vi "getSerializedData.vi"(0 "reference in":refnum<class "DQMHModuleNode.lvclass">, 5 "error in (no error)":errorcluster) -> (14 "reference out":refnum<class "DQMHModuleNode.lvclass">, 15 "parent":refnum<class "AbstractNode.lvclass">, 16 "children":refnum<class "AbstractNode.lvclass">[](array[class]), 17 "xmlOut":string, 19 "error out":errorcluster)   [LabVIEW 2020, in "DQMHModuleNode.lvclass"]
doc: "Gets data to store"
uses:
  <resource>/Framework/Providers/Open_GDS/UML/DQMHModuleNode_class/DQMHModuleNode.lvclass
  C:/Program Files (x86)/National Instruments/LabVIEW 2020/resource/Framework/Providers/Open_GDS/UML/AbstractNode_class/AbstractNode.lvclass
  C:/Program Files (x86)/National Instruments/LabVIEW 2020/resource/Framework/Providers/Open_GDS/UML/RectangularNode_class/RectangularNode.lvclass
  <resource>/Framework/Providers/Open_GDS/UML/AbstractNode_class/AbstractNode.lvclass
  <resource>/Framework/Providers/Open_GDS/UML/MultiLineString_class/MultiLineString.lvclass
  <resource>/Framework/Providers/Open_GDS/UML/RectangularNode_class/RectangularNode.lvclass
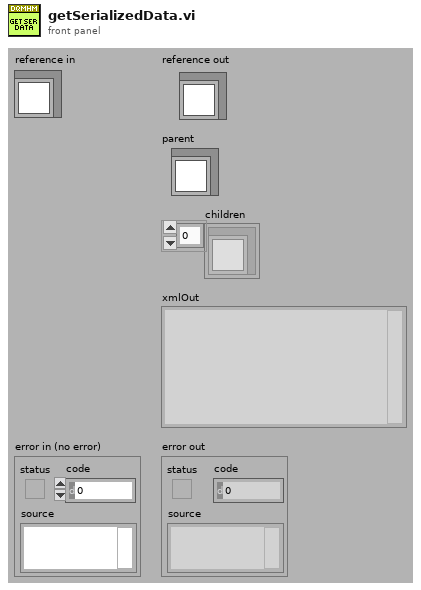
[diagram p1: front panel]
types:
  T1 = typedef "AbstractNode.lvclass/ObjectAttributes.ctl" = cluster{"parent":refnum<class "AbstractNode.lvclass">, "children":refnum<class "AbstractNode.lvclass">[], "Hidden":bool}
  T2 = typedef "RectangularNode.lvclass/ObjectAttributes.ctl" = cluster{"bounds":T3}
  T3 = typedef "Rectangle Rectangle2D.ctl" = cluster{"x":dbl, "y":dbl, "width":dbl, "height":dbl}
  T4 = typedef "DQMHModuleNode.lvclass/ObjectAttributes.ctl" = cluster{"DescriptionHeight":dbl, "InternalDataHeight":dbl, "EventsHeight":dbl, "Name":refnum<class "MultiLineString.lvclass">, "Description":refnum<class "MultiLineString.lvclass">, "InternalData":refnum<class "MultiLineString.lvclass">, "Events":refnum<class "MultiLineString.lvclass">, "showDescription":bool, "showInternalData":bool, "showEvents":bool, "DEFAULT_ROUNDING":i32, "DEFAULT_WIDTH":i32, "DEFAULT_HEIGHT":i32, "ClassPath":path, "Template":string, "Icon":u8[][]}
  T5 = cluster{"data string":string, "text":string, "text":string, "text":string, "text":string}
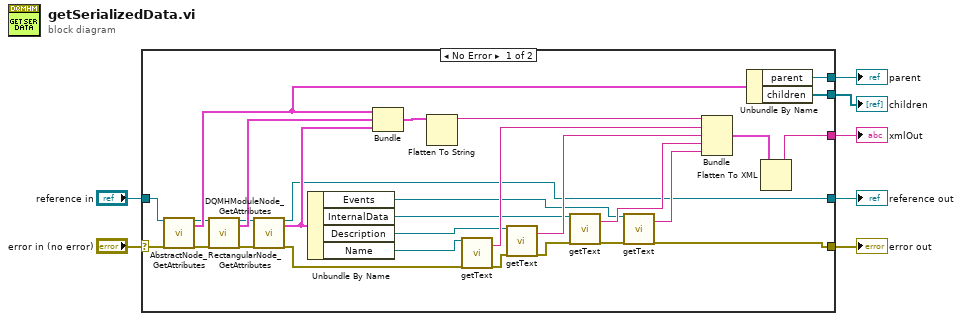
[diagram p0: block diagram]
diagram:
  n1 = case shown="No Error" "error in (no error)" {
    selector: "error in (no error)" -> [w15 w37]
    tunnel: "reference in" -> [w14 w38]
    tunnel: [w26 w37] -> w5
    tunnel: [w10 w38] -> w4
    tunnel: [w36 _] -> w3
    tunnel: [w35 _] -> w2
    tunnel: [w34 _] -> w1
    frame No Error {
      n2 = call <resource>:"AbstractNode_GetAttributes.vi"("reference in"=w14, "error in (no error)"=w15) -> ("reference out"=w12:refnum<class "DQMHModuleNode.lvclass">, "Data"=w20:T1, "error out"=w16:errorcluster)  [unwired: 14 in, 1 out]
      n3 = call <resource>:"RectangularNode_GetAttributes.vi"("reference in"=w12, "error in (no error)"=w16) -> ("reference out"=w13:refnum<class "DQMHModuleNode.lvclass">, "Data"=w19:T2, "error out"=w17:errorcluster)  [unwired: 14 in, 1 out]
      n4 = call <resource>:"DQMHModuleNode_GetAttributes.vi"("reference in"=w13, "error in (no error)"=w17) -> ("reference out"=w10:refnum<class "DQMHModuleNode.lvclass">, "Data"=w18:T4, "error out"=w11:errorcluster)  [unwired: 1 in, 14 out]
      n5 = Unbundle By Name(w18) -> ("Events"=w22:refnum<class "MultiLineString.lvclass">, "InternalData"=w23:refnum<class "MultiLineString.lvclass">, "Description"=w24:refnum<class "MultiLineString.lvclass">, "Name"=w25:refnum<class "MultiLineString.lvclass">)
      n6 = Bundle("Data"=w20, "Data"=w19, "Data"=w18) -> (w9:cluster{"Data":T1, "Data":T2, "Data":T4})  [unwired: 1 in]
      n7 = Flatten To String(anything=w9) -> (data string=w8:string)  [unwired: 3 in, 2 out]
      n8 = call-dynamic "getText.vi"("reference"=w25, "error in (no error)"=w11) -> ("text"=w30:string, "error out"=w31:errorcluster)  [unwired: 16 out]
      n9 = call-dynamic "getText.vi"("reference"=w24, "error in (no error)"=w31) -> ("text"=w29:string, "error out"=w32:errorcluster)  [unwired: 16 out]
      n10 = call-dynamic "getText.vi"("reference"=w23, "error in (no error)"=w32) -> ("text"=w28:string, "error out"=w27:errorcluster)  [unwired: 16 out]
      n11 = call-dynamic "getText.vi"("reference"=w22, "error in (no error)"=w27) -> ("text"=w21:string, "error out"=w26:errorcluster)  [unwired: 16 out]
      n12 = Bundle("data string"=w8, "text"=w30, "text"=w29, "text"=w28, "text"=w21) -> (w33:T5)  [unwired: 1 out]
      n13 = Unbundle By Name(w20) -> ("parent"=w36:refnum<class "AbstractNode.lvclass">, "children"=w35:refnum<class "AbstractNode.lvclass">[])
      n14 = Flatten To XML(6:w33) -> (2:w34:string)
    }
    frame Error {
    }
  }
  "reference out" <- w4
  "error out" <- w5
  "children" <- w2
  "parent" <- w3
  "xmlOut" <- w1
